vi "VIH ExtCmd - Send Build Status Response.vi"(4 "Errors":i32, 6 "Help Info file":path, 8 "error in":errorcluster, 9 "CHM file":path, 10 "HHP file":path, 11 "HTML Build Log file":path) -> (0 "error out":errorcluster)   [LabVIEW 2014]
doc: "::: VI Helpeks :::\nCopyright (c) 2000-2026 Konstantin Shifershteyn. All rights reserved."
panel:
  # "VI Helpeks\nCopyright (c) 2012-2026 Konstantin Shifershteyn"
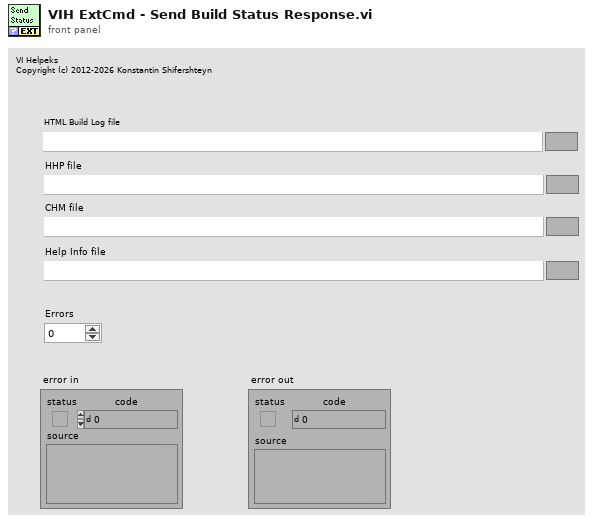
[diagram p1: front panel]
types:
  T1 = cluster{"Msg":string, "Data":string, "error":errorcluster}
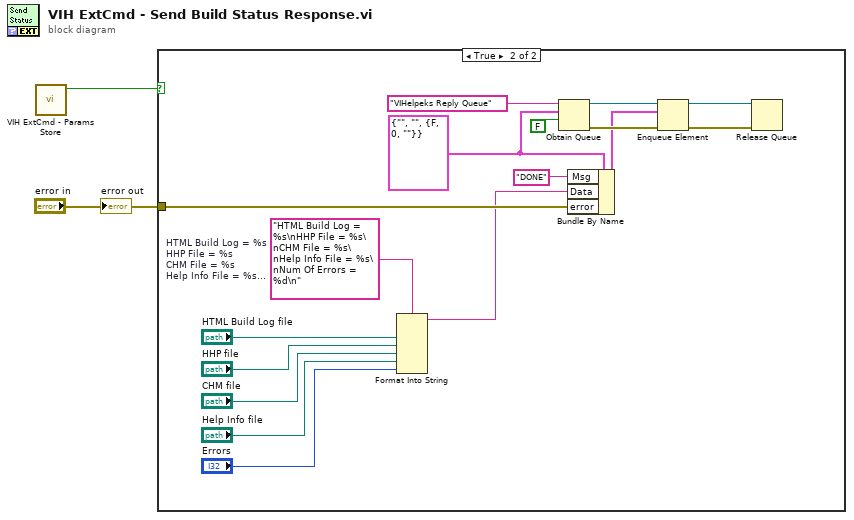
[diagram p0: block diagram]
diagram:
  n1 = call "VIH ExtCmd - Params Store.vi"() -> ("Ext Command"=w1:bool)  [unwired: 10 in, 1 out]
  n2 = case shown="True" w1 {
    tunnel: "error in" -> [_ w11]
    frame False {
    }
    frame True {
      w9 = "HTML Build Log = %s\nHHP File = %s\nCHM File = %s\nHelp Info File = %s\nNum Of Errors = %d\n"  # HTML Build Log = %s HHP File = %s CHM File = %s Help Info File = %s Num Of Errors = %d
      w15 = T1 {"Msg"="", "Data"="", "error"={"status"=FALSE, "code"=0, "source"=""}}
      n3 = Format Into String(format string=w9, "HTML Build Log file", "HHP file", "CHM file", "Help Info file", "Errors") -> (resulting string=w7:string)  [unwired: 2 in, 1 out]
      n4 = Obtain Queue(name (unnamed)="VIHelpeks Reply Queue", element data type=w15, create if not found? (T)=FALSE) -> (queue out=w17:refnum<queue>, error out=w16:errorcluster)  [unwired: 2 in, 1 out]
      n5 = Bundle By Name(cluster=w15, "Msg"="DONE", "Data"=w7, "error"=w11) -> (w10:T1)
      n6 = Enqueue Element(queue=w17, element=w10, error in (no error)=w16) -> (queue out=w14:refnum<queue>, error out=w13:errorcluster)  [unwired: 1 in, 1 out]
      n7 = Release Queue(queue=w14, error in (no error)=w13) -> ()  [unwired: 1 in, 3 out]
    }
  }
  "error out" <- "error in"
